vi "Ximea get frame and display.vi"(8 "error in (no error)":errorcluster, 10 "Image In":T1, 11 "xiCam In":refnum<k24>) -> (0 "error out":errorcluster, 1 "FrameNumber":u32, 2 "Image Out":T1, 3 "xiCam Out":refnum<k24>)   [LabVIEW 2016]
uses:
  C:/Users/Ries Lab/Documents/Microscope Control from Sheng Account/Microscope-Control/Device Library/Cameras/Ximea/xiLIB_64bit/xiLIB/xiCamLib/API/x64/xiApi.NETX64.dll
  xiLIB_64bit/xiLIB/xiCamLib/API/x64/xiApi.NETX64.dll
  <vilib>/vision/Image Controls.llb/IMAQ Image.ctl
  Camera Controls/Camera IMAQ Key Info.ctl
  xiLIB_64bit/xiLIB/xiCamLib/xiCam/Utils/xiImageManager/xiImageMng - State.ctl
  xiLIB_64bit/xiLIB/xiCamLib/xiCam/PRM/PRM/PRM_v2.ctl
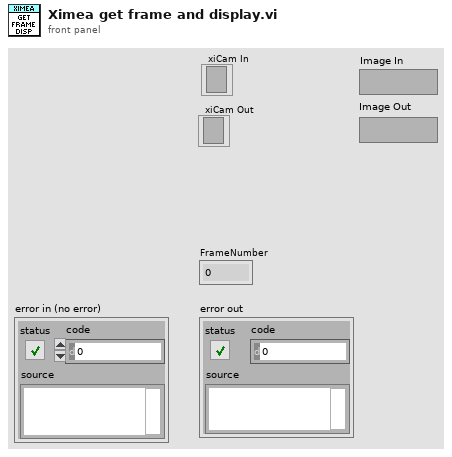
[diagram p1: front panel]
types:
  T1 = typedef "IMAQ Image.ctl" = refnum<image>
  T2 = typedef "PRM_v2.ctl" = enum16{"ACQ_BUFFER_SIZE", "ACQ_FRAME_BURST_COUNT", "ACQ_TIMING_MODE", "ACQ_TRANSPORT_BUFFER_SIZE", "AE_MAX_LIMIT", "AEAG", "AEAG_LEVEL", "API_VERSION", "AG_MAX_LIMIT", "APPLY_CMS", "AUTO_BANDWIDTH_CALCULATION", "AUTO_WB", "AVAILABLE_BANDWIDTH", "AVAILABLE_BANDWIDTH_MAX", "AVAILABLE_BANDWIDTH_MIN", "BUFFER_POLICY", "BUFFERS_QUEUE_SIZE", "CC_MATRIX_00", "CC_MATRIX_01", "CC_MATRIX_02", "CC_MATRIX_03", "CC_MATRIX_10", "CC_MATRIX_11", "CC_MATRIX_12", "CC_MATRIX_13", "CC_MATRIX_20", "CC_MATRIX_21", "CC_MATRIX_22", "CC_MATRIX_23", "CC_MATRIX_30", "CC_MATRIX_31", "CC_MATRIX_32", "CC_MATRIX_33", "CHIP_TEMP", "CMS", "COLOR_FILTER_ARRAY", "COOLING", "DEBOUNCE_EN", "DEBOUNCE_POL", "DEBOUNCE_T0", "DEBOUNCE_T1", "DEBUG_LEVEL", "DEFAULT_CC_MATRIX", "DEVICE_INSTANCE_PATH", "DEVICE_MODEL_ID", "DEVICE_NAME", "DEVICE_SN", "DEVICE_TYPE", "DEVICE_USER_ID", "DOWNSAMPLING", "DOWNSAMPLING_TYPE", "DRV_VERSION", "EXP_PRIORITY", "EXPOSURE", "EXPOSURE_MAX", "EXPOSURE_MIN", "FFS_FILE_NAME", "FPGA1_VERSION", "FRAMERATE", "FRAMERATE_MAX", "FRAMERATE_MIN", "FREE_FFS_SIZE", "GAIN", "GAIN_MAX", "GAIN_MIN", "GAMMAC", "GAMMAY", "GPI_LEVEL", "GPI_MODE", "GPI_SELECTOR", "GPO_MODE", "GPO_SELECTOR", "HDR", "HDR_T1", "HDR_T2", "HEIGHT", "HEIGHT_MAX", "HEIGHT_MIN", "HOUSE_TEMP", "IMAGE_DATA_FORMAT", "IMAGE_IS_COLOR", "INPUT_CMS_PROFILE", "IS_COOLED", "IS_DEVICE_EXIST", "KNEEPOINT1", "KNEEPOINT2", "LED_MODE", "LED_SELECTOR", "LIMIT_BANDWIDTH", "LIMIT_BANDWIDTH_MAX", "LIMIT_BANDWIDTH_MIN", "LUT_EN", "LUT_INDEX", "LUT_INDEX_MAX", "LUT_INDEX_MIN", "LUT_VALUE", "LUT_VALUE_MAX", "LUT_VALUE_MIN", "MANUAL_WB", "MCU1_VERSION", "MCU2_VERSION", "OFFSET_X", "OFFSET_X_MAX", "OFFSET_X_MIN", "OFFSET_Y", "OFFSET_Y_MAX", "OFFSET_Y_MIN", "OUTPUT_CMS_PROFILE", "OUTPUT_DATA_BIT_DEPTH", "OUTPUT_DATA_PACKING", "READ_FILE_FFS", "RECENT_FRAME", "SENSOR_DATA_BIT_DEPTH", "SENSOR_MODE", "SENSOR_TAPS", "SHARPNESS", "SHUTTER_TYPE", "TARGET_TEMP", "TRG_DELAY", "TRG_SELECTOR", "TRG_SOFTWARE", "TRG_SOURCE", "USED_FFS_SIZE", "WB_KB", "WB_KG", "WB_KR", "WIDTH", "WIDTH_MAX", "WIDTH_MIN", "WRITE_FILE_FFS", "ACQ_BUFFER_SIZE_UNIT", "ACQ_TRANSPORT_BUFFER_COMMIT", "AEAG_ROI_HEIGHT", "AEAG_ROI_OFFSET_X", "AEAG_ROU_OFFSET_Y", "AEAG_ROI_WIDTH", "API_CONTEXT_LIST", "BINNING_HORIZONTAL", "BINNING_SELECTOR", "BINNING_VERTICAL", "COLUMN_FPN_CORRECTION", "COUNTER_SELECTOR", "COUNTER_VALUE", "DECIMATION_HORIZONTAL", "DECIMATION_SELECTOR", "DECIMATION_VERTICAL", "DEVICE_ID", "DEVICE_LOCATION_PATH", "DEVICE_MANIFEST", "DEVICE_RESET", "DEVICE_SENS_SN", "EXPOSURE_BURST_COUNT", "FFS_ACCESS_KEY", "GAIN_SELECTOR", "HW_REVISION", "IMAGE_BLACK_LEVEL", "IMAGE_DATA_BIT_DEPTH", "IMAGE_DATA_FORMAT_RGB32_ALPHA", "IMAGE_PAYLOAD_SIZE", "LENS_APERTURE_VALUE", "LENS_FEATURE", "LENS_FEATURE_SELECTOR", "LENS_FOCAL_LENGTH", "LENS_FOCUS_DISTANCE", "LENS_FOCUS_MOVE", "LENS_FOCUS_MOVEMENT_VALUE", "LENS_MODE", "OUTPUT_DATA_PACKING_TYPE", "SENSOR_CLOCK_FREQ_HZ", "SENSOR_CLOCK_FREQ_INDEX", "SENSOR_FEATURE_SELECTOR", "SENSOR_FEATURE_VALUE", "SENSOR_OUTPUT_CHANNEL_COUNT", "TRANSPORT_PIXEL_FORMAT", "TS_RST_MODE", "TS_RST_SOURCE", "SENS_DEFECTS_CORR_LIST_SELECTOR", "SENS_DEFECTS_CORR", "SENS_DEFECTS_CORR_LIST_CONTENT", "DEVICE_UNIT_SELECTOR", "DEVICE_UNIT_REGISTER_SELECTOR", "DEVICE_UNIT_REGISTER_VALUE"}
  T3 = typedef "xiImageMng - State.ctl" = enum16{"Init", "GetProperties", "SetProperties"}
  T4 = typedef "Camera IMAQ Key Info.ctl" = cluster{"Frame":u32, "Sensor Height":i32, "Sensor Width":i32, "ROI Height":i32, "ROI Width":i32, "ROI Enable?":bool, "Bit per Pixel":u8}
  T5 = typedef "xiImageMng - Attributes.ctl" = cluster{"WIDTH":i32, "HEIGHT":i32, "IMG_FORMAT":T6}
  T6 = typedef "IMG_DATA_FORMAT.ctl" = enum16{"MONO8", "MONO16", "RGB24", "RGB32", "RGBPLANAR", "RAW8", "RAW16"}
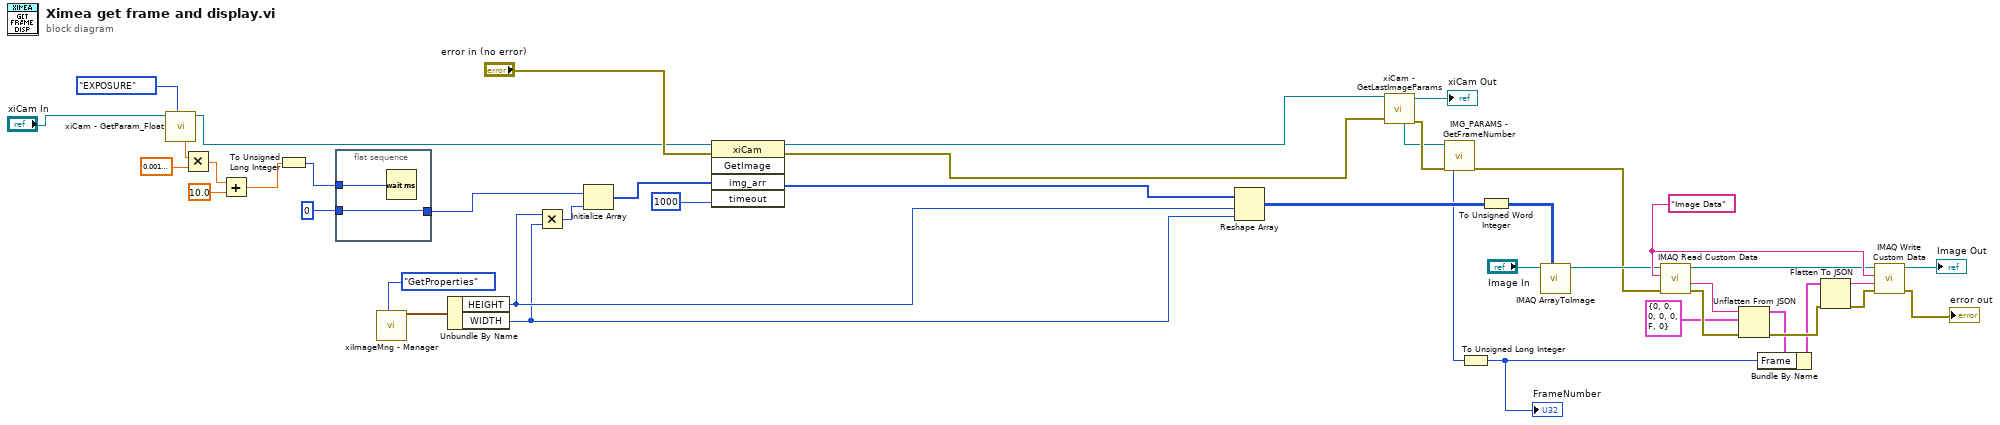
[diagram p0: block diagram]
diagram:
  w40 = "Image Data" ("Key")
  n1 = call "xiCam - GetParam_Float.vi"("PRM"=PRM_v2."EXPOSURE", "xiCam In"="xiCam In") -> ("xiCam Out"=w4:refnum<k24>, "Float_Value"=w7:sgl)  [unwired: 7 in, 1 out]
  n2 = Multiply(x=w7, y=sgl 0.001) -> (x*y=w3:sgl)
  n3 = Add(x=w3, y=sgl 10.0) -> (x+y=w1:sgl)
  n4 = To Unsigned Long Integer(number=w1) -> (unsigned 32bit integer=w6:u32)
  n5 = flat-sequence {
    tunnel: [w46] -> w10
    tunnel: u8 0 ("element") -> [w46]
    tunnel: w6 -> [w45]
    frame #0 {
      n6 = Wait (ms)(milliseconds to wait=w45) -> ()  [unwired: 1 out]
    }
  }
  n7 = call "xiImageMng - Manager.vi"("State"=xiImageMng_-_State."GetProperties") -> ("Properties Out"=w21:T5)  [unwired: 9 in, 1 out]
  n8 = Unbundle By Name(w21) -> ("HEIGHT"=w15:i32, "WIDTH"=w14:i32)
  n9 = Multiply(x=w15, y=w14) -> (x*y=w20:i32)
  n10 = Initialize Array(w10, w20) -> (w19:u8[])
  n11 = invoke class="xiCam" method="GetImage"(reference=w4, error in="error in (no error)", "img_arr"=w19, "timeout"=1000) -> (reference out=w12:refnum<k24>, error out=w13:errorcluster, "img_arr"=w16:u8[])  [unwired: 1 in, 2 out]
  n12 = Reshape Array(w16, w15, w14) -> (w31:u8[][])
  n13 = call "xiCam - GetLastImageParams.vi"("error in (no error)"=w13, "xiCam In"=w12) -> ("error out"=w24:errorcluster, "xiCam Out"=→"xiCam Out":refnum<k24>, "GetLastImageParams"=w23:refnum<k24>)  [unwired: 7 in]
  n14 = call "IMG_PARAMS - GetFrameNumber.vi"("error in (no error)"=w24, "xiApi.NET.ImgParams"=w23) -> ("error out"=w26:errorcluster, "FrameNumber"=w25:i32)  [unwired: 7 in, 1 out]
  n15 = To Unsigned Long Integer(number=w25) -> (unsigned 32bit integer=w32:u32)
  "FrameNumber" <- w32
  n16 = To Unsigned Word Integer(number=w31) -> (unsigned 16bit integer=w30:u16[][])
  n17 = call "IMAQ ArrayToImage"("Image Pixels (U16)"=w30, "Image"="Image In") -> ("Image Out"=w28:T1)  [unwired: 8 in, 1 out]
  n18 = call "IMAQ Read Custom Data"("error in (no error)"=w26, "Key"=w40, "Image"=w28) -> ("error out"=w41:errorcluster, "Custom Data Out"=w36:string, "Image (duplicate)"=w34:T1)  [unwired: 6 in]
  n19 = Unflatten From JSON(JSON string=w36, type and defaults=T4 {"Frame"=0, "Sensor Height"=0, "Sensor Width"=0, "ROI Height"=0, "ROI Width"=0, "ROI Enable?"=FALSE, "Bit per Pixel"=0} ("Camera IMAQ Key Info"), error in (no error)=w41) -> (value=w37:T4, error out=w42:errorcluster)  [unwired: 4 in]
  n20 = Bundle By Name(cluster=w37, "Frame"=w32) -> (w38:T4)
  n21 = Flatten To JSON(anything=w38, error in (no error)=w42) -> (JSON string=w39:string, 11:w43:errorcluster)  [unwired: 1 in]
  n22 = call "IMAQ Write Custom Data"("error in (no error)"=w43, "Custom Data In"=w39, "Key"=w40, "Image"=w34) -> ("error out"=→"error out":errorcluster, "Image Out"=→"Image Out":T1)  [unwired: 6 in]
